vi "_CoercionTest.vi"(0 "VI Reference In":refnum<vi>, 5 "Subpanel Details":string, 11 "error in":errorcluster) -> (4 "VI Reference Out":refnum<vi>, 15 "error out":errorcluster)   [LabVIEW 2016, in "SubpanelTests.lvlib"]
doc: "Coercison test"
uses:
  SubpanelTests.lvlib
  APIs/Stimulus/KeyBoardSimulation/KeyBoardSimulationForTargetVI.vi
  APIs/Assert/AssertControlValue/Equal.vi
  <vilib>/addons/_JKI Toolkits/Caraya/classes/Test/Test.lvclass
  Drona.lvlib
  APIs/Stimulus/KeyBoardSimulation/KeyboardSimulation.lvlib
  APIs/Assert/AssertControlValue/AssertControlValue.lvlib
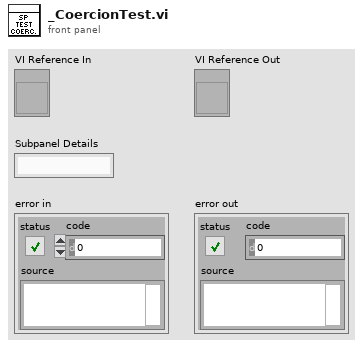
[diagram p1: front panel]
types:
  T1 = cluster{"Test Label":string, "Key In Array":cluster{" Key":u8, "Action":enum16{"Press", "Up", "Down"}, "Delay (ms)":u32}[], "Assert Value":dbl}[]
  T2 = cluster{" Key":u8, "Action":enum16{"Press", "Up", "Down"}, "Delay (ms)":u32}[]
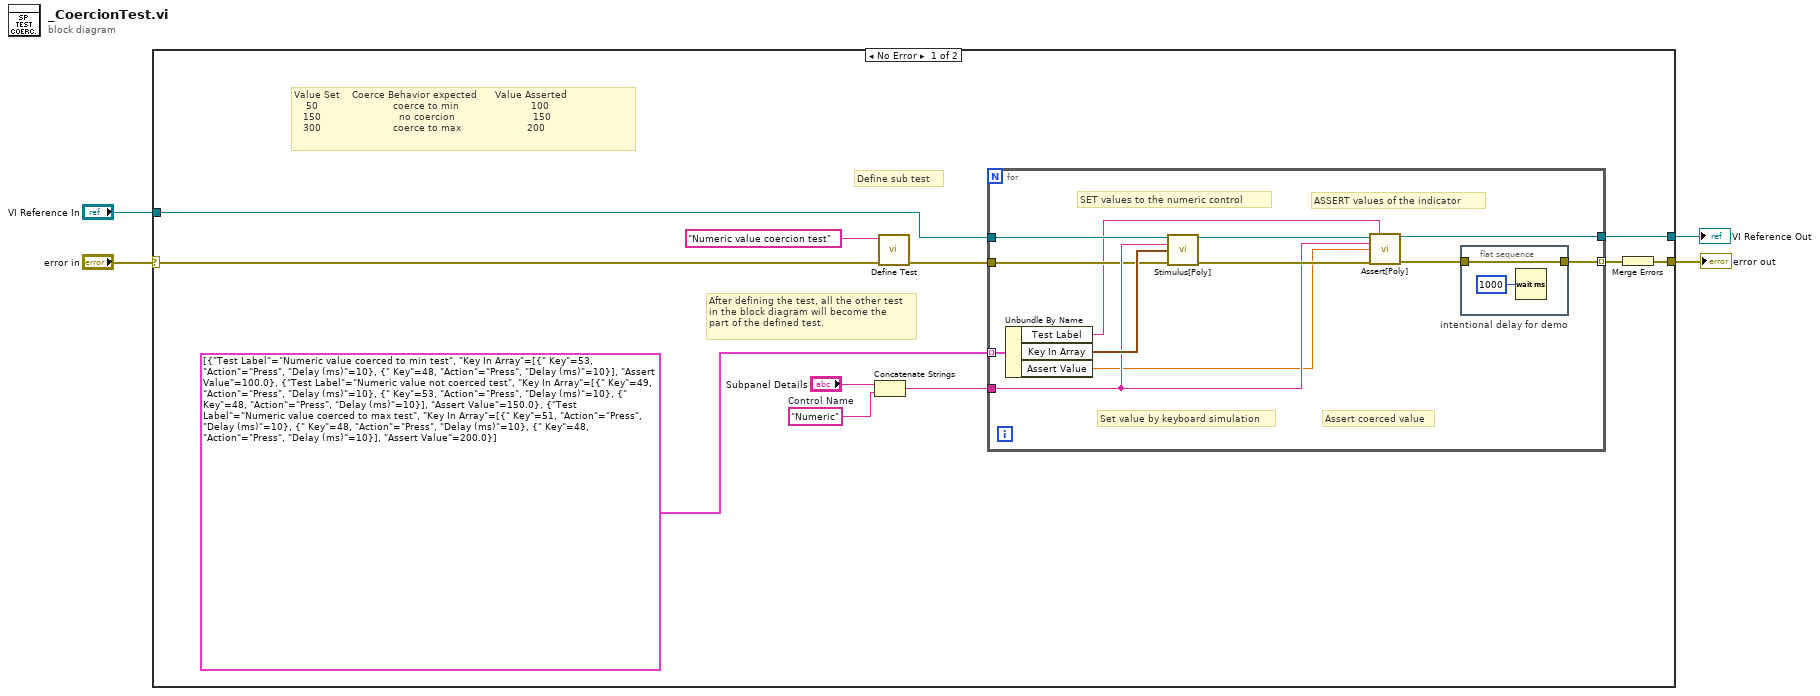
[diagram p0: block diagram]
diagram:
  n1 = case shown="No Error" "error in" {
    selector: "error in" -> [w15 w30]
    tunnel: "VI Reference In" -> [w9 w31]
    tunnel: [w6 w31] -> w2
    tunnel: [w5 w30] -> w1
    frame No Error {
      w12 = "Numeric"  # Control Name
      # "Value Set    Coerce Behavior expected      Value Asserted\n    50                         coerce to min                        100\n   150                          no coercion                          150\n   300                        coerce to max                      200"
      # "After defining the test, all the other test\nin the block diagram will become the \npart of the defined test."
      # "Define sub test"
      n2 = Concatenate Strings("Subpanel Details", w12) -> (w11:string)
      n3 = call <vilib>:"Define Test.vi"("error in (no error)"=w15, "Label (VI Title)"="Numeric value coercion test") -> ("error out"=w7:errorcluster)  [unwired: 8 in, 1 out]
      n4 = for {
        tunnel: T1 [{"Test Label"="Numeric value coerced to min test", "Key In Array"=[{" Key"=53, "Action"=enum."Press", "Delay (ms)"=10}, {" Key"=48, "Action"=enum."Press", "Delay (ms)"=10}], "Assert Value"=100.0}, {"Test Label"="Numeric value not coerced test", "Key In Array"=[{" Key"=49, "Action"=enum."Press", "Delay (ms)"=10}, {" Key"=53, "Action"=enum."Press", "Delay (ms)"=10}, {" Key"=48, "Action"=enum."Press", "Delay (ms)"=10}], "Assert Value"=150.0}, {"Test Label"="Numeric value coerced to max test", "Key In Array"=[{" Key"=51, "Action"=enum."Press", "Delay (ms)"=10}, {" Key"=48, "Action"=enum."Press", "Delay (ms)"=10}, {" Key"=48, "Action"=enum."Press", "Delay (ms)"=10}], "Assert Value"=200.0}] -> [w27] mode=indexing
        tunnel: w11 -> [w23]
        tunnel: w9 -> [w22]
        tunnel: w7 -> [w21]
        tunnel: [w19] -> w8 mode=indexing
        tunnel: [w16] -> w6
        # "Set value by keyboard simulation"
        # "Assert coerced value"
        # "ASSERT values of the indicator"
        # "SET values to the numeric control"
        n5 = Unbundle By Name(w27) -> ("Test Label"=w17:string, "Key In Array"=w24:T2, "Assert Value"=w18:dbl)
        n6 = call-poly "Stimulus[Poly].vi"("VI Reference In"=w22, "Control Path"=w23, "Key Array"=w24, "error In"=w21) -> ("VI Reference Out"=w25:refnum<vi>, "error IO"=w26:errorcluster)  [unwired: 10 in]
        n7 = call-poly "Assert[Poly].vi"("VI Reference In"=w25, "Test Label"=w17, "Control Path"=w23, "Control Value"=w18, "Error In"=w26) -> ("VI Reference Out"=w16:refnum<vi>, "Error Out"=w20:errorcluster)  [unwired: 8 in, 1 out]
        n8 = flat-sequence "intentional delay for demo" {
          tunnel: w20 -> [w28]
          tunnel: [w28] -> w19
          frame #0 {
            n9 = Wait (ms)(milliseconds to wait=u32 1000) -> ()  [unwired: 1 out]
          }
        }
      }
      n10 = Merge Errors(w8) -> (w5:errorcluster)
    }
    frame Error {
    }
  }
  "error out" <- w1
  "VI Reference Out" <- w2
